vi "check folder on off VI.vi"(8 "エラー入力":errorcluster, 9 "selected EX":string[](array[string]), 10 "folder names":string[](array[string]), 11 "M_selectioninput":u16(ring) items=["AXN1", "AXN2", "AXN3", "AXN4", "AXN5", "AXN6", "AXN7", "AXN8", "C_Local", "D_Local"]) -> (0 "error out":errorcluster, 1 "Array 4":string[](array[string]), 3 "Array 3":cluster{string, bool}[](array[cluster]))   [LabVIEW 2018]
panel:
  out "M_selection_List":string[](array[string])
  out "M_selectioninput 2":u16(ring) items=["AX1", "AX2", "AX3", "AXN1", "AXN2", "AX3", "AXN4", "AXN5", "AXN6", "AXN7", "AXN3"]
  out "size(s) 2":i32
  out "Array 2":string[](array[string])
  out "Array":string[](array[string])
  out "size(s)":i32
  out "Up Table":string[][](table) caption="Read Table"
  out "stripped path":path
  out "path":path
  out "ex_path":path
  out "100k_path":path
  out "10k_path":path
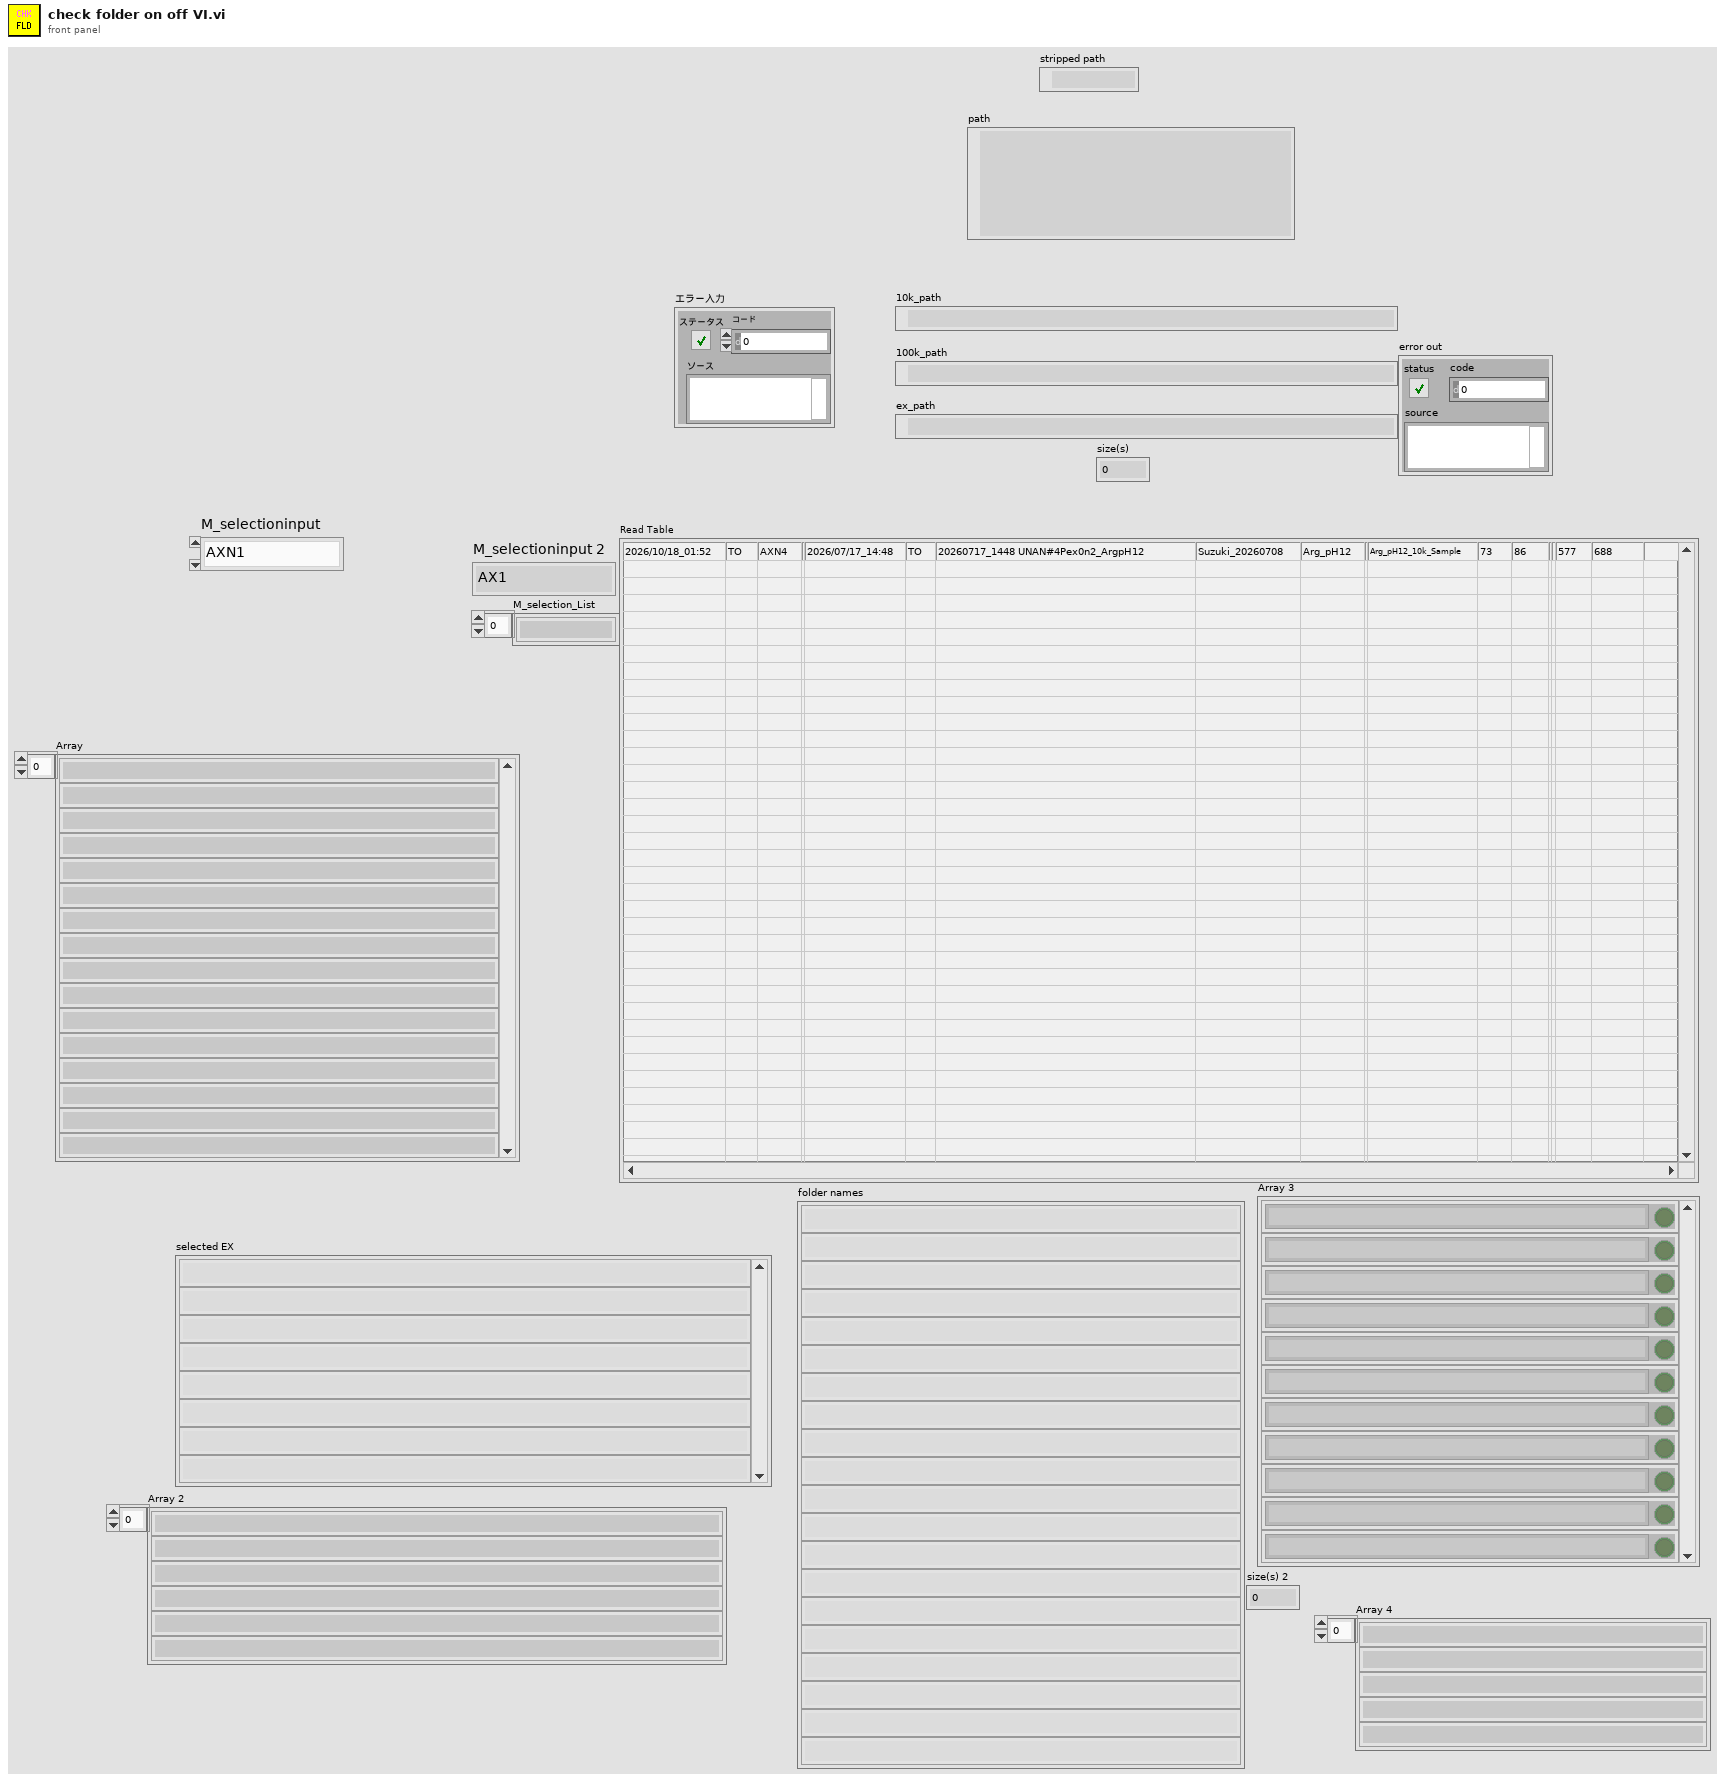
[diagram p1: front panel]
types:
  T1 = enum16{"open", "replace", "create", "open or create", "replace or create", "replace or create with confirmation"}
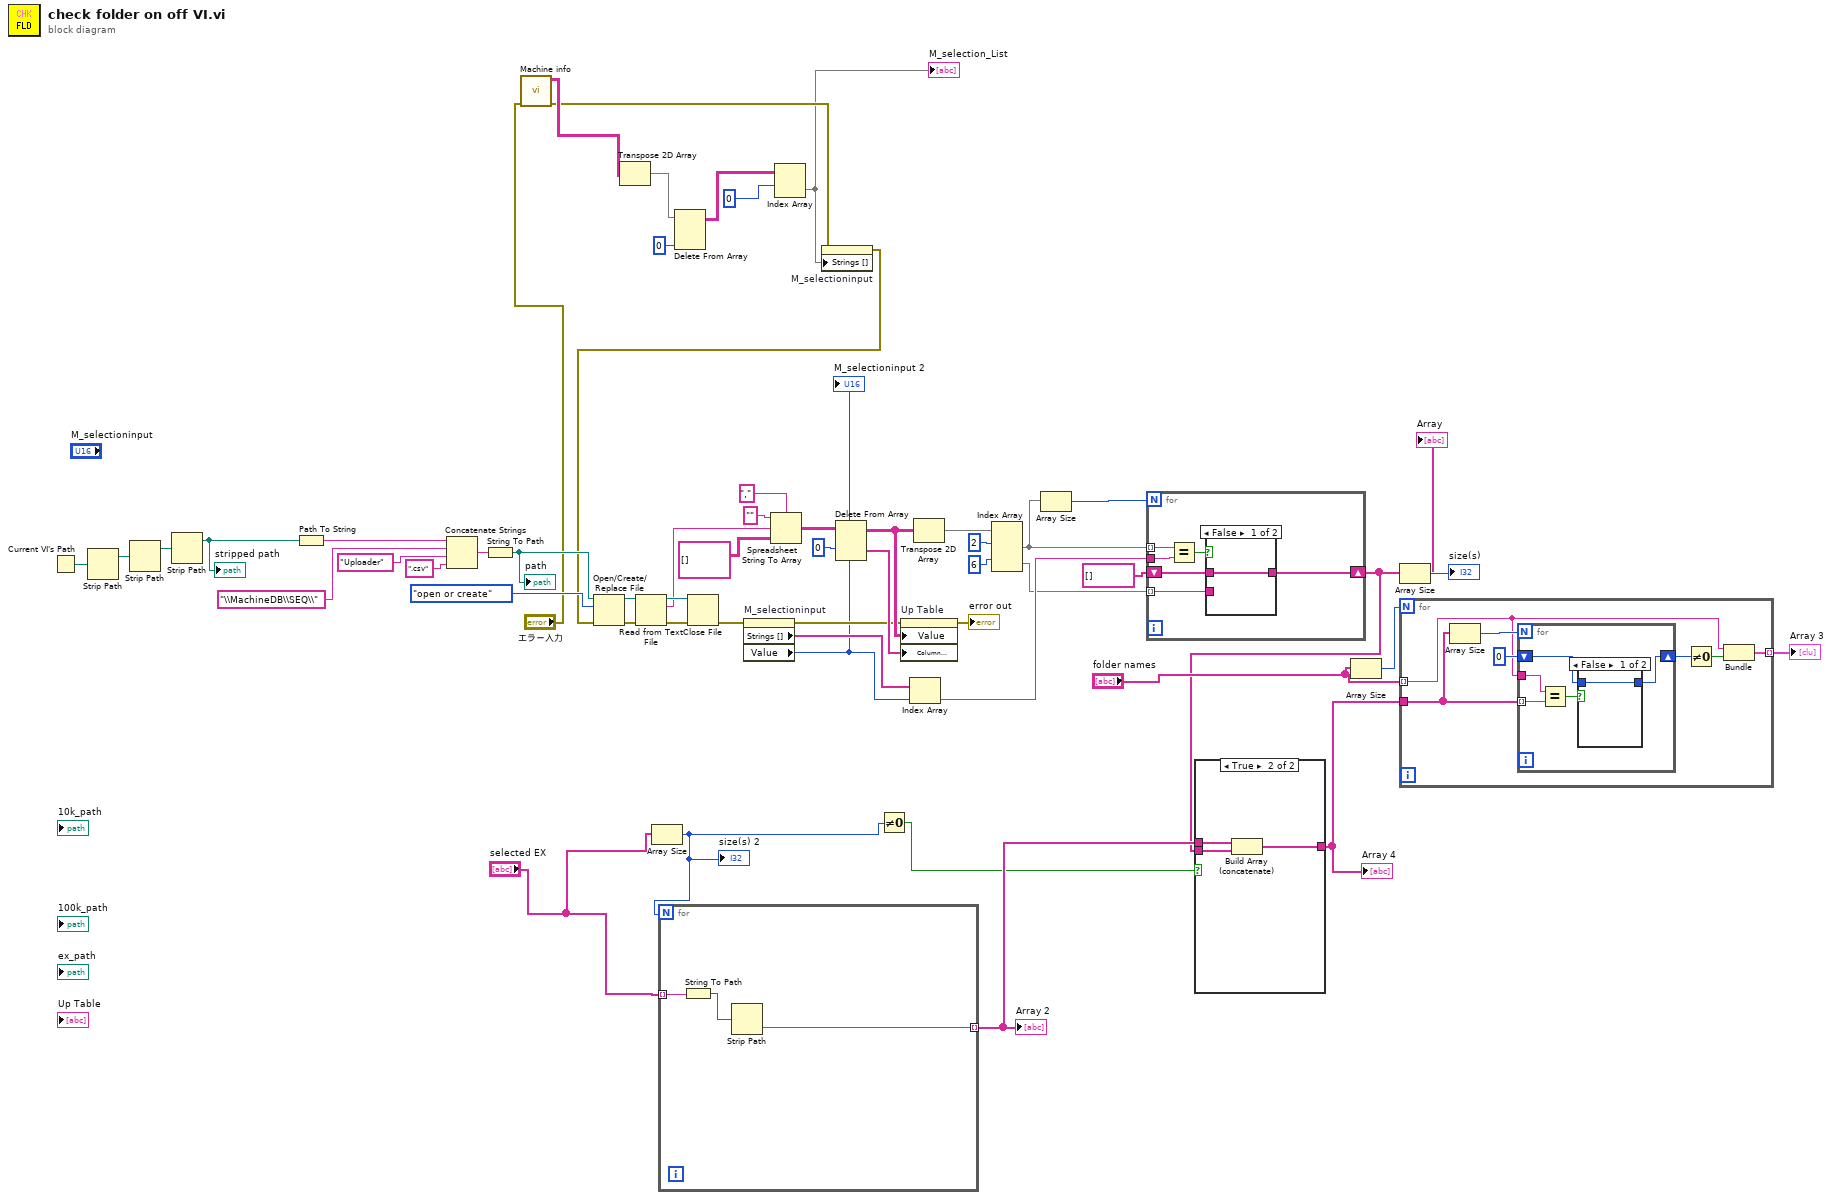
[diagram p0: block diagram]
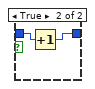
[diagram p3: hidden frame]
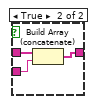
[diagram p4: hidden frame]
diagram:
  n1 = Current VI's Path() -> (path=w40:path)
  n2 = Strip Path(path=w40) -> (stripped path=w39:path)  [unwired: 1 out]
  n3 = Strip Path(path=w39) -> (stripped path=w38:path)  [unwired: 1 out]
  n4 = Strip Path(path=w38) -> (stripped path=w37:path)  [unwired: 1 out]
  "stripped path" <- w37
  n5 = Path To String(path=w37) -> (string=w45:string)
  n6 = Concatenate Strings(w45, "\\MachineDB\\SEQ\\" ("string"), "Uploader" ("string"), ".csv" ("文字列")) -> (w42:string)
  n7 = String To Path(string=w42) -> (path=w50:path)
  "path" <- w50
  n8 = call "Machine info.vi"("error in"="エラー入力") -> ("error out"=w3:errorcluster, "transposed array"=w5:string[][])  [unwired: 9 in]
  n9 = Transpose 2D Array(2D array=w5) -> (transposed array=w8:string[][])
  n10 = Array Size(array="selected EX") -> (size(s)=w14:i32)
  "size(s) 2" <- w14
  n11 = for {
    N: w14 -> [_]
    tunnel: "selected EX" -> [w58] mode=indexing
    tunnel: [w56] -> w15 mode=indexing
    n12 = String To Path(string=w58) -> (path=w57:path)
    n13 = Strip Path(path=w57) -> (name=w56:string)  [unwired: 1 out]
  }
  "Array 2" <- w15
  n14 = Delete From Array(array=w8, index (col)=0 ("disabled index (col)")) -> (array with subset deleted=w7:string[][])  [unwired: 2 in, 1 out]
  n15 = Index Array(array=w7, index (row)=0) -> (element=w1:string[])  [unwired: 1 in]
  "M_selection_List" <- w1
  n16 = property on="M_selectioninput" class="Ring (strict)"(error in=w3, "Strings []"=w1) -> (error out=w2:errorcluster)  [unwired: 1 in, 1 out]
  n17 = Open/Create/Replace File(file path (use dialog)=w50, error in=w2, operation (0:open)=T1."open or create" ("操作（0:open）")) -> (refnum out=w54:refnum<file>, error out=w55:errorcluster)  [unwired: 3 in, 1 out]
  n18 = Read from Text File(file (use dialog)=w54, error in=w55) -> (refnum out=w51:refnum<file>, text=w47:string, error out=w52:errorcluster)  [unwired: 2 in, 1 out]
  n19 = Close File(refnum=w51, error in=w52) -> (error out=w26:errorcluster)  [unwired: 1 out]
  n20 = property on="M_selectioninput" class="Ring (strict)"(error in=w26) -> (error out=w25:errorcluster, "Strings []"=w24:string[], "Value"=w23:u16)  [unwired: 1 in, 1 out]
  "M_selectioninput 2" <- w23
  n21 = Spreadsheet String To Array(delimiter (Tab)="," ("デリミタ（タブ）"), format string="" ("形式文字列"), spreadsheet string=w47, array type (2D Dbl)=string[][] [] ("付加配列")) -> (array=w33:string[][])
  n22 = Delete From Array(array=w33, index (row)=0) -> (deleted portion=w34:string[], array with subset deleted=w30:string[][])  [unwired: 2 in]
  n23 = Not Equal To 0?(x=w14) -> (x != 0?=w13:bool)
  n24 = property on="Up Table" class="Tbl (strict)"(error in=w25, "Value"=w30, "Column Headers[]"=w34) -> (error out=→"error out":errorcluster)  [unwired: 1 in, 1 out]
  n25 = Index Array(array=w24, index=w23) -> (element=w22:string)
  n26 = Transpose 2D Array(2D array=w30) -> (transposed array=w32:string[][])
  n27 = Index Array(array=w32, index (row) #1=2 ("index (row)"), index (row) #2=6 ("index (row)")) -> (element #1=w27:string[], element #2=w21:string[])  [unwired: 2 in]
  n28 = Array Size(array=w27) -> (size(s)=w28:i32)
  n29 = for {
    N: w28 -> [_]
    tunnel: w27 -> [w64] mode=indexing
    tunnel: w22 -> [w63]
    tunnel: w21 -> [w61] mode=indexing
    shift-right: [w60] -> w11
    shift-left: string[] [] -> [w59]
    n30 = Equal?(x=w64, y=w63) -> (x = y?=w62:bool)
    n31 = case shown="False" w62 {
      tunnel: w61 -> [_ w68]
      tunnel: [w65 w67] -> w60
      tunnel: w59 -> [w65 w66]
      frame False {
      }
      frame True {
        n32 = Build Array (concatenate)(w66, w68) -> (w67:string[])
      }
    }
  }
  "Array" <- w11
  n33 = case shown="True" w13 {
    tunnel: w15 -> [_ w72]
    tunnel: w11 -> [w69 w71]
    tunnel: [w69 w70] -> w10
    frame False {
    }
    frame True {
      n34 = Build Array (concatenate)(w72, w71) -> (w70:string[])
    }
  }
  "Array 4" <- w10
  n35 = Array Size(array="folder names") -> (size(s)=w18:i32)
  n36 = Array Size(array=w11) -> (size(s)=→"size(s)":i32)
  n37 = for {
    N: w18 -> [_]
    tunnel: w10 -> [w78]
    tunnel: "folder names" -> [w74] mode=indexing
    tunnel: [w73] -> w17 mode=indexing
    n38 = Array Size(array=w78) -> (size(s)=w79:i32)
    n39 = for {
      N: w79 -> [_]
      tunnel: w74 -> [w84]
      tunnel: w78 -> [w83] mode=indexing
      shift-right: [w81] -> w76
      shift-left: 0 -> [w80]
      n40 = Equal?(x=w84, y=w83) -> (x = y?=w82:bool)
      n41 = case shown="False" w82 {
        tunnel: [w85 w87] -> w81
        tunnel: w80 -> [w85 w86]
        frame False {
        }
        frame True {
          n42 = Increment(x=w86) -> (x+1=w87:i32)
        }
      }
    }
    n43 = Not Equal To 0?(x=w76) -> (x != 0?=w75:bool)
    n44 = Bundle(w74, w75) -> (w73:cluster{string, bool})  [unwired: 1 in]
  }
  "Array 3" <- w17
